vi "Measurement Logic.vi"() -> ()   [LabVIEW 2021, in "Ripple_PMIC.lvlib"]
uses:
  Ripple_PMIC.lvlib
  <vilib>/Plug-In SDKs/Measurements/Measure Call Context/Measure Call Context.lvclass
  Measurement Results.ctl
  Measurement Configuration.ctl
  <instrlib>/niDCPower/nidcpower.llb/niDCPower Output Function.ctl
  <instrlib>/niDCPower/nidcpower.llb/niDCPower Source Mode.ctl
  <instrlib>/niDCPower/nidcpower.llb/niDCPower Wait For Event - Event.ctl
  <instrlib>/niDCPower/nidcpower.llb/niDCPower Measurement Type.ctl
  <instrlib>/niScope/Controls/niScope vertical coupling.ctl
  <instrlib>/niScope/Controls/niScope trigger slope.ctl
  <instrlib>/niScope/Controls/niScope trigger coupling.ctl
  <instrlib>/niScope/Controls/niScope timestamp type.ctl
  <instrlib>/niScope/Configure/Trigger/niScope Configure Trigger Edge.vi
  <instrlib>/niScope/Acquire/Fetch/niScope Fetch WDT.vi
  <vilib>/measure/madcrms.llb/Basic Averaged DC-RMS for 1 Chan.vi
  <vilib>/Plug-In SDKs/Measurements/Measure Call Context/Accessor/Is Canceled.vi
  <instrlib>/niDCPower/nidcpower.llb/niDCPower Get Channel Name From String.vi
  <vilib>/measure/NI_MAPro.lvlib
panel:
  in  "measurement configuration":T1={"Mode of operation"=enum."Perform measurement", "DUT setup time"=0.005, "Aperture time"=0.005, "Source resource name"="", "Source sense"=1009, "Source voltage level"=10.0, "Source current limit"=15.0, "Load resource name"="", "Load sense"=1009, "Load current level"=6.0, "Load voltage limit range"=6.0, "Scope resource name"="", "Scope channel name"="0", "Scope sample rate"=10000.0, "Scope acquisition time"=3.0, "Scope probe attenuation"=1.0} {"Load sense" items=["Local"=1008, "Remote"=1009]; "Source sense" items=["Local"=1008, "Remote"=1009]}
  out "measurement results":T2
  out "measure call context out":refnum<class "Measure Call Context.lvclass">
  in  "measure call context in":refnum<class "Measure Call Context.lvclass">
  out "error out":errorcluster
  in  "error in":errorcluster
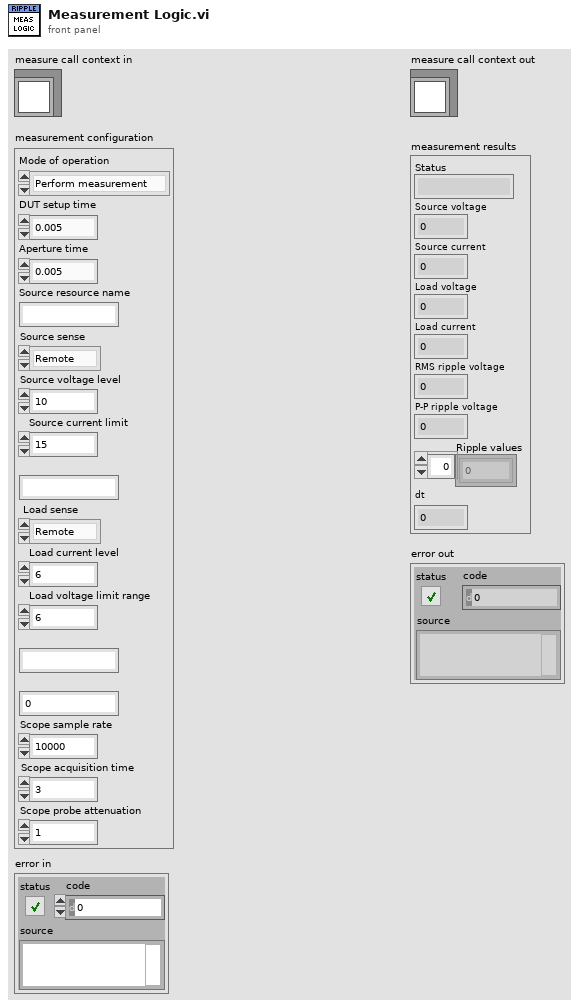
[diagram p1: front panel]
types:
  T1 = typedef "Ripple_PMIC.lvlib/Measurement Configuration.ctl" = cluster{"Mode of operation":enum32{"Power on the DUT", "Perform measurement", "Power off the DUT"}, "DUT setup time":dbl, "Aperture time":dbl, "Source resource name":string, "Source sense":i32, "Source voltage level":dbl, "Source current limit":dbl, "Load resource name":string, "Load sense":i32, "Load current level":dbl, "Load voltage limit range":dbl, "Scope resource name":string, "Scope channel name":string, "Scope sample rate":dbl, "Scope acquisition time":dbl, "Scope probe attenuation":dbl}
  T2 = typedef "Ripple_PMIC.lvlib/Measurement Results.ctl" = cluster{"Status":string, "Source voltage":dbl, "Source current":dbl, "Load voltage":dbl, "Load current":dbl, "RMS ripple voltage":dbl, "P-P ripple voltage":dbl, "Ripple values":dbl[], "dt":dbl}
  T3 = cluster{"Source Session":refnum<k15>, "Load Session":refnum<k15>, "Scope Session":refnum<k15>, "Source channel":string, "Load channel":string}
  T4 = enum32{"Power on the DUT", "Perform measurement", "Power off the DUT"}
  T5 = typedef "niDCPower Wait For Event - Event.ctl" = i32
  T6 = typedef "niDCPower Source Mode.ctl" = i32
  T7 = typedef "niDCPower Output Function.ctl" = i32
  T8 = typedef "niDCPower Measurement Type.ctl" = i32
  T9 = typedef "niScope trigger coupling.ctl" = u16
  T10 = typedef "niScope trigger slope.ctl" = i32
  T11 = typedef "niScope vertical coupling.ctl" = i32
  T12 = typedef "niScope timestamp type.ctl" = i32
  T13 = cluster{"actualSamples":i32, "absoluteInitialX":dbl, "relativeInitialX":dbl, "xIncrement":dbl, "offset":dbl, "gain":dbl, "reserved1":dbl, "reserved2":dbl}
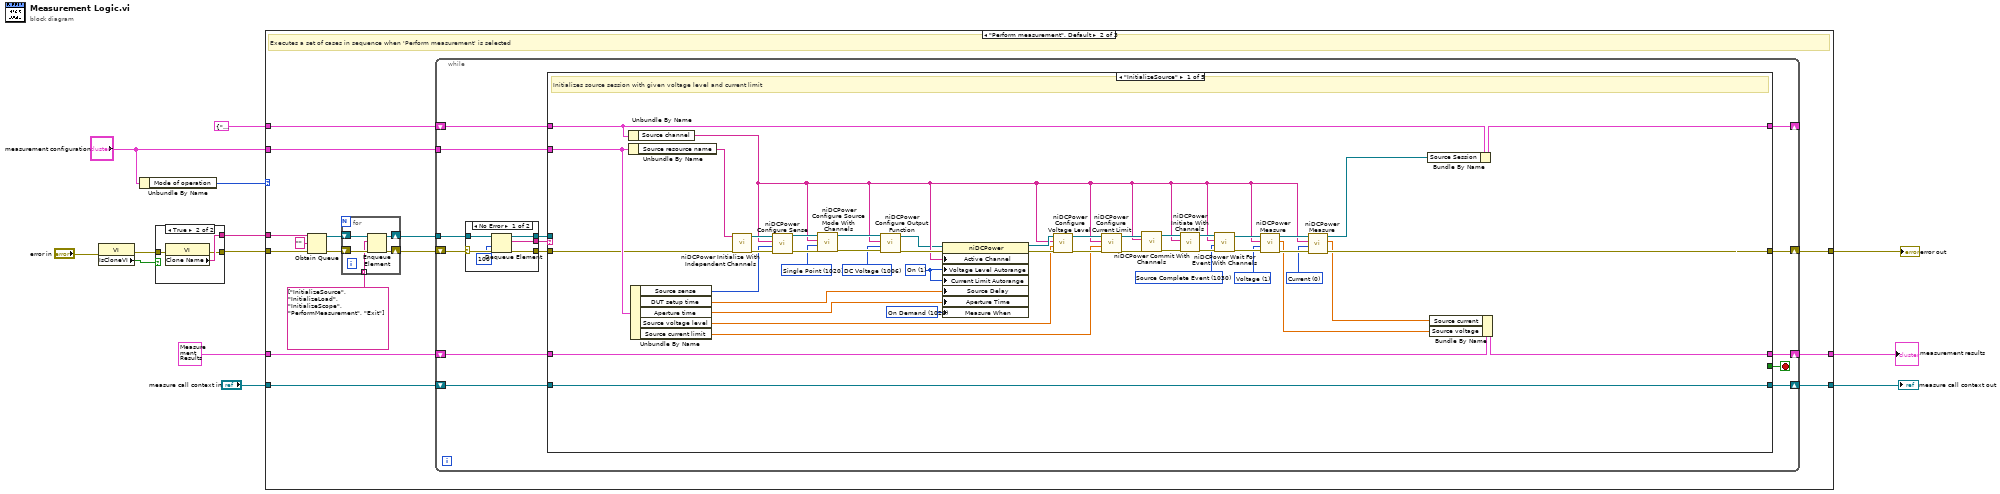
[diagram p0: block diagram]
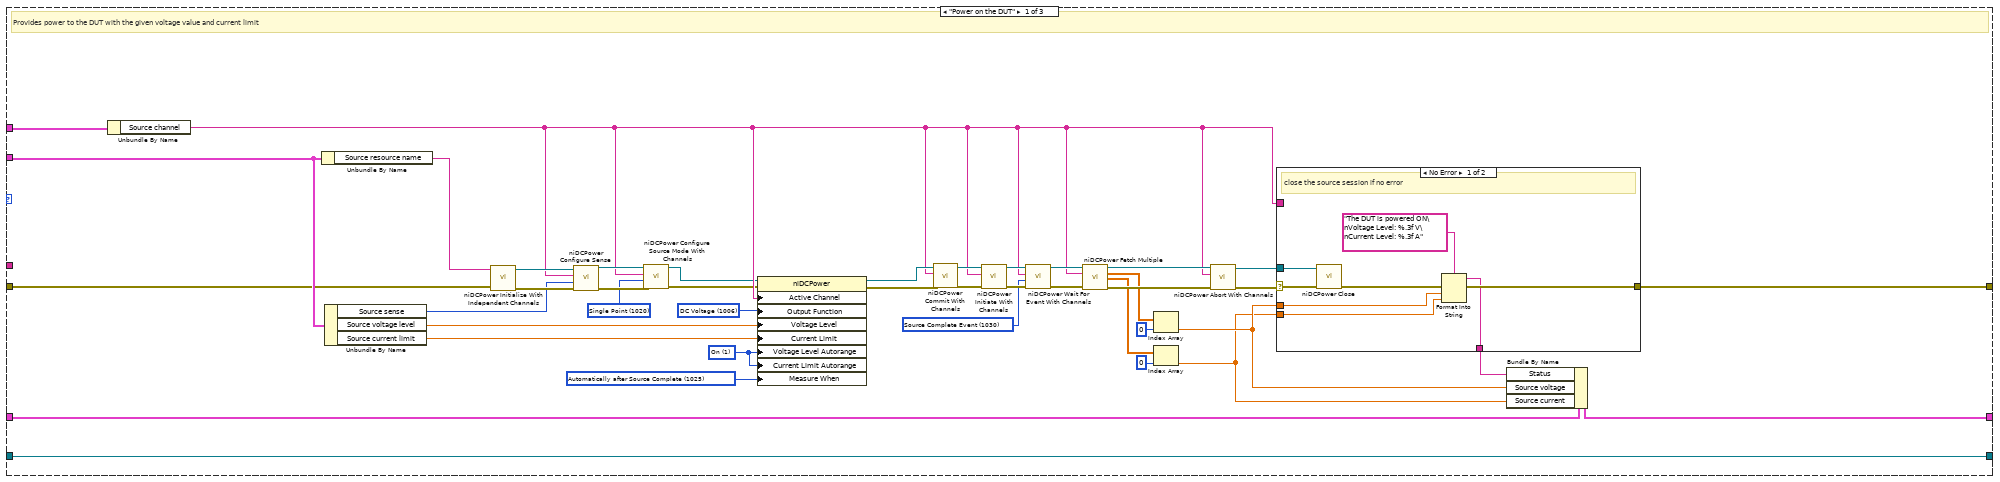
[diagram p2: hidden frame]
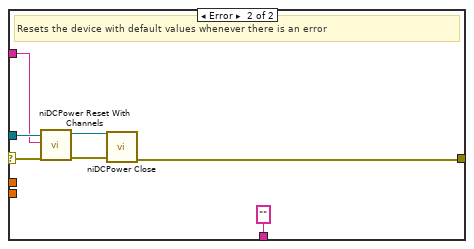
[diagram p3: hidden frame]
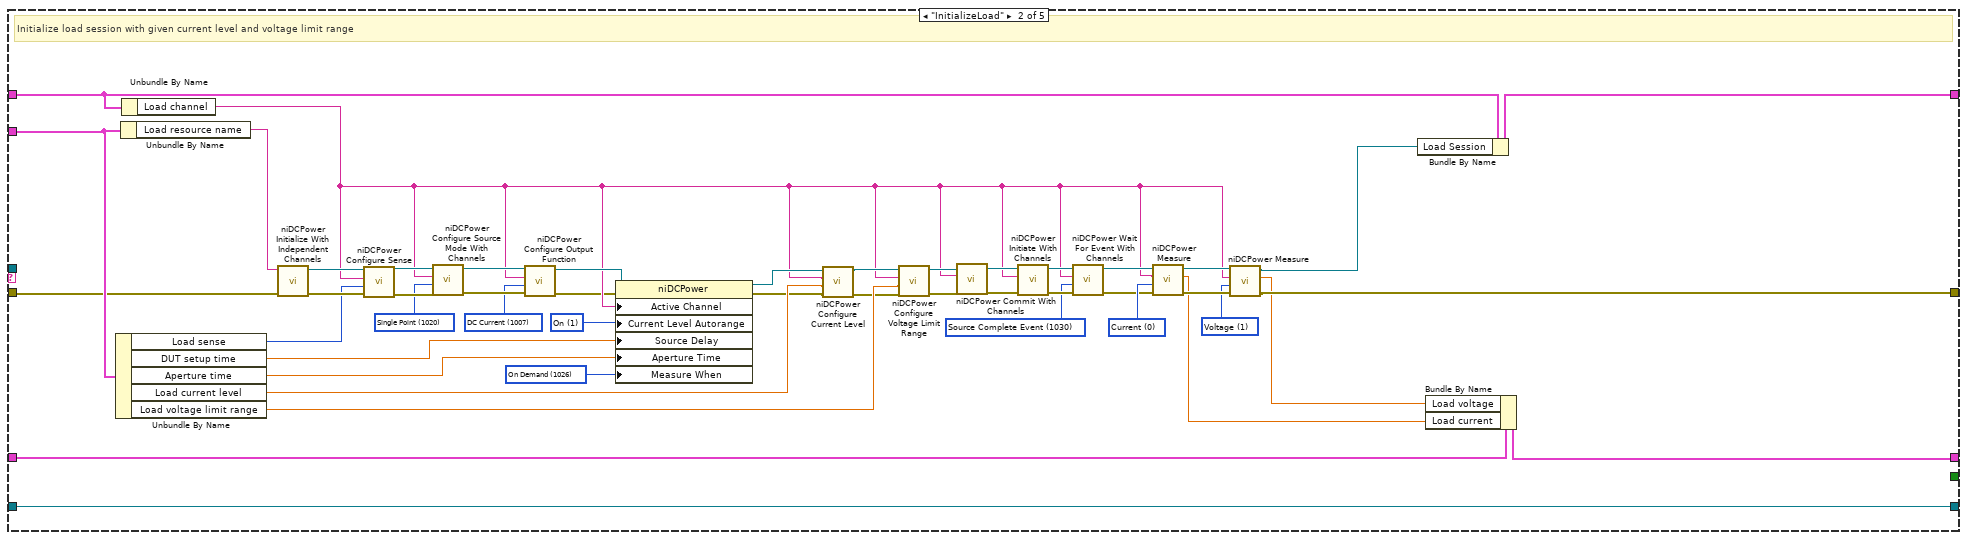
[diagram p4: hidden frame]
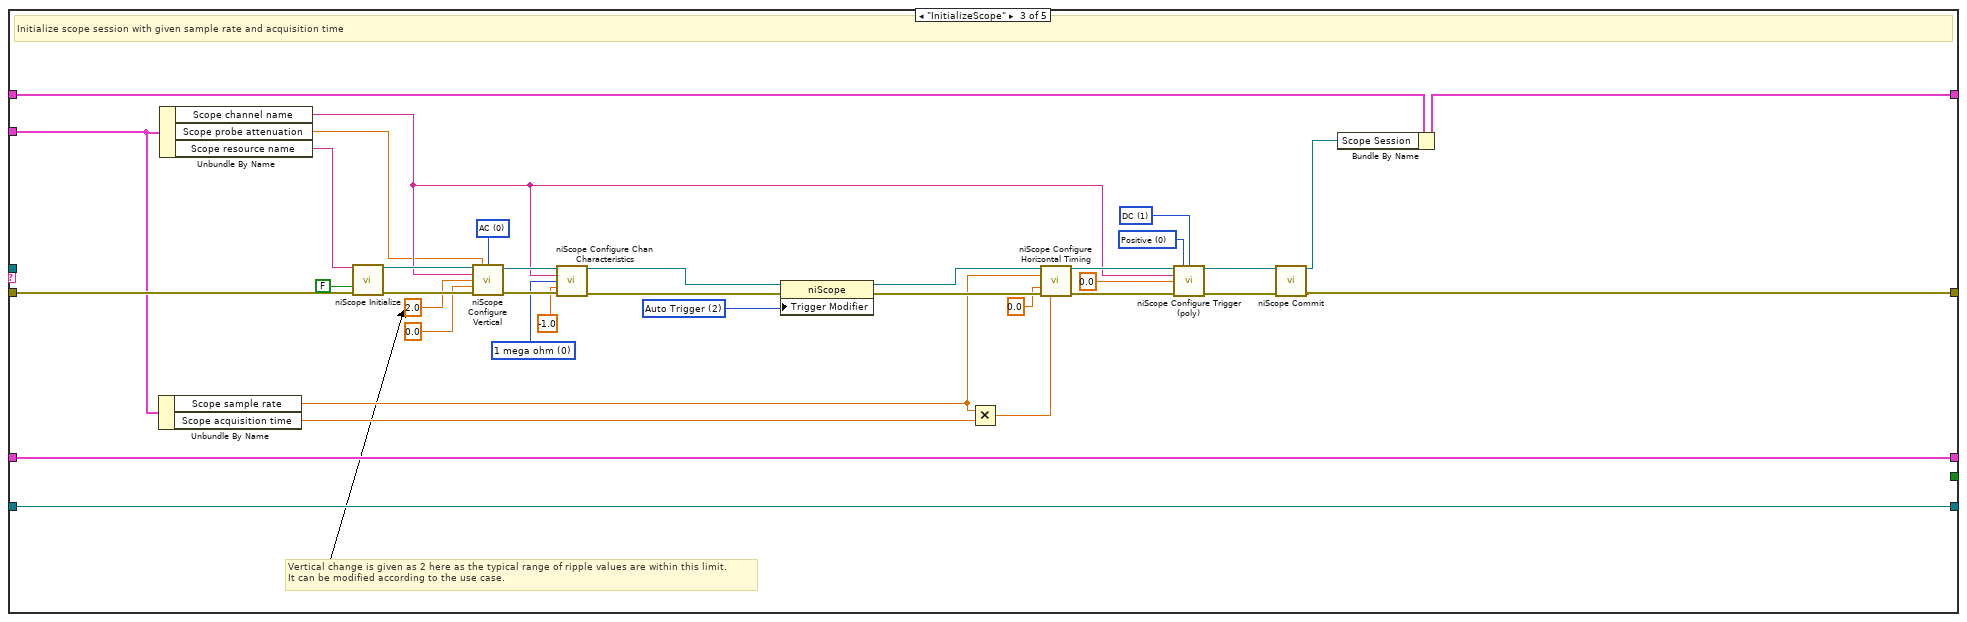
[diagram p5: hidden frame]
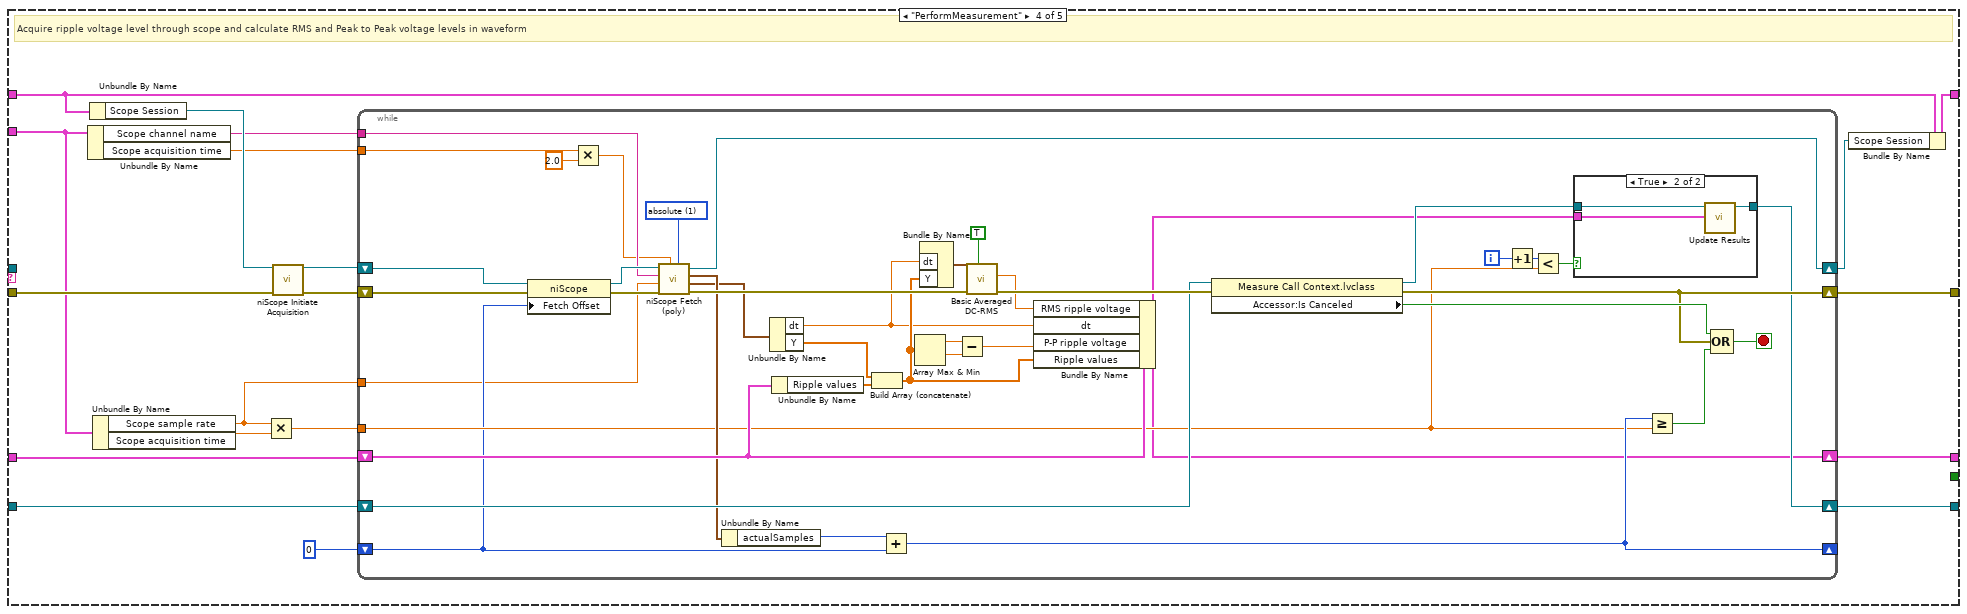
[diagram p6: hidden frame]
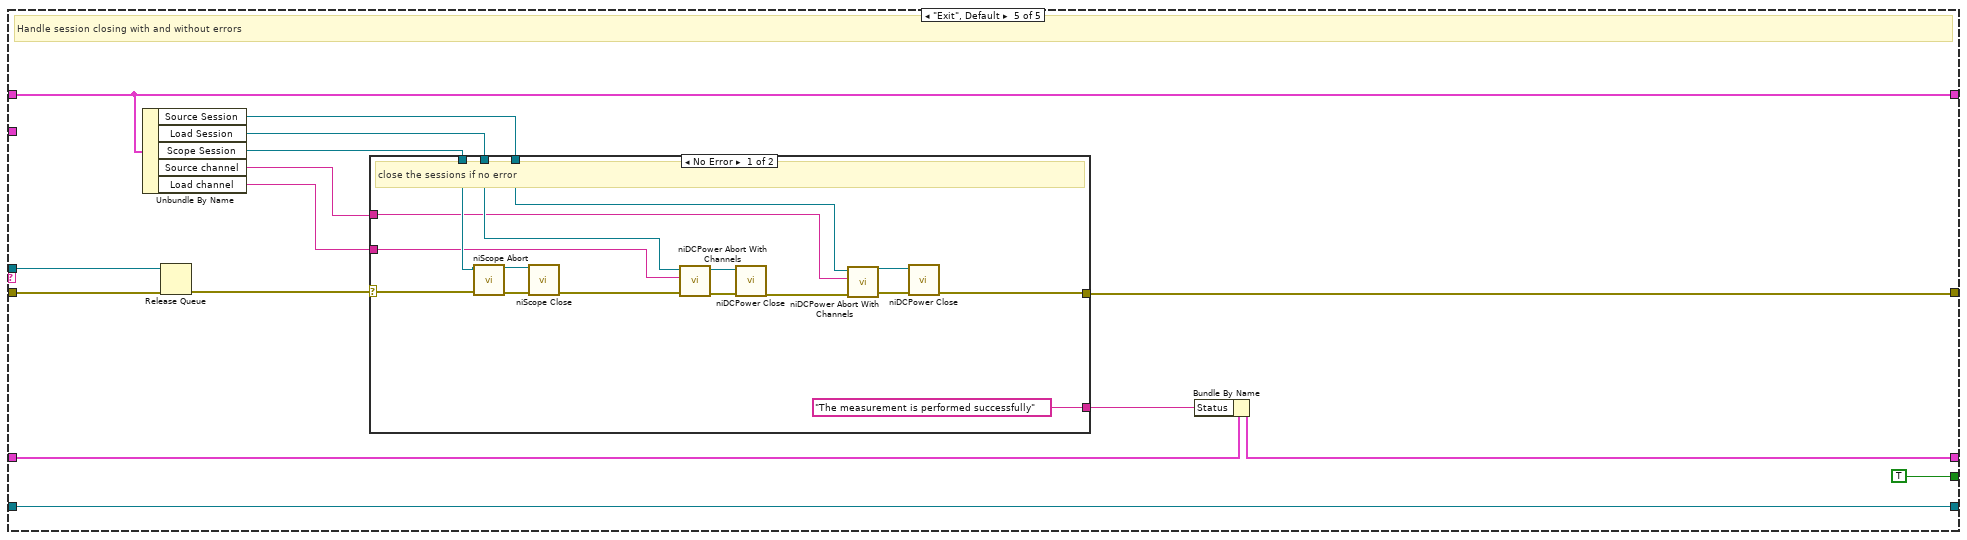
[diagram p8: hidden frame]
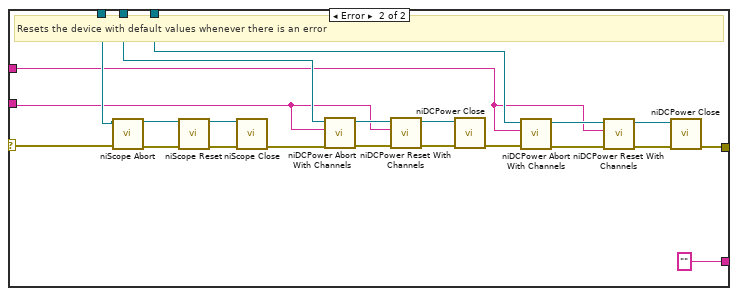
[diagram p9: hidden frame]
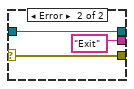
[diagram p10: hidden frame]
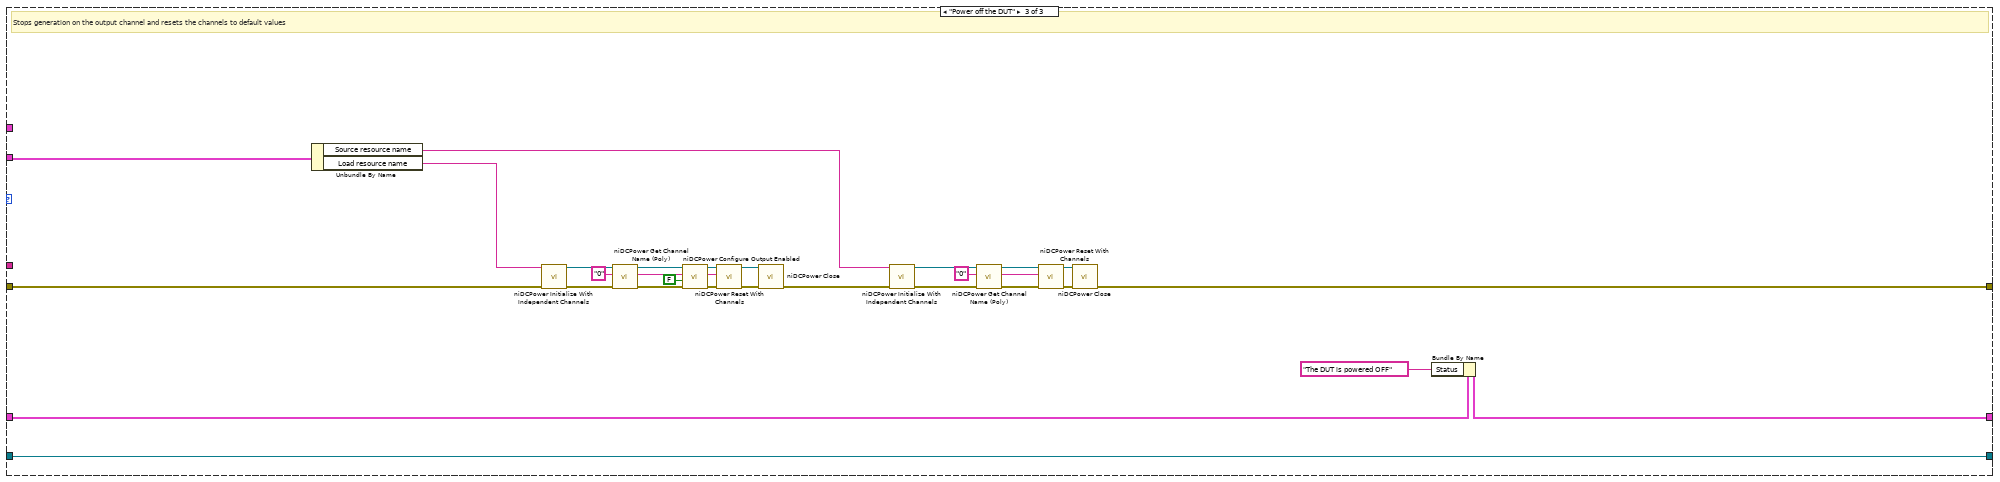
[diagram p11: hidden frame]
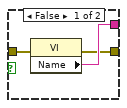
[diagram p12: hidden frame]
diagram:
  n1 = property class="VI"(error in="error in") -> (error out=w12:errorcluster, "IsCloneVI"=w13:bool)  [unwired: 1 in, 1 out]
  n2 = Unbundle By Name("measurement configuration") -> ("Mode of operation"=w6:T4)
  n3 = case shown="True" w13 {
    tunnel: w12 -> [w16 w19]
    tunnel: [w15 w18] -> w4
    tunnel: [w14 w17] -> w5
    frame False {
      n4 = property class="VI"(error in=w16) -> (error out=w14:errorcluster, "Name"=w15:string)  [unwired: 1 in, 1 out]
    }
    frame True {
      n5 = property class="VI"(error in=w19) -> (error out=w17:errorcluster, "Clone Name"=w18:string)  [unwired: 1 in, 1 out]
    }
  }
  n6 = case shown="\"Perform measurement\", Default" w6 {
    tunnel: T3 {"Source Session"="", "Load Session"="", "Scope Session"="", "Source channel"="0", "Load channel"="0"} ("Cluster") -> [w41 w91 _]
    tunnel: T2 {"Status"="", "Source voltage"=0.0, "Source current"=0.0, "Load voltage"=0.0, "Load current"=0.0, "RMS ripple voltage"=0.0, "P-P ripple voltage"=0.0, "Ripple values"=[], "dt"=0.0} ("Measurement Results") -> [w44 w90 w371]
    tunnel: [w39 w89 w375] -> w8
    tunnel: "measurement configuration" -> [w46 w88 w376]
    tunnel: [w45 w87 w370] -> w7
    tunnel: w5 -> [w40 w81 w374]
    tunnel: w4 -> [_ w80 _]
    tunnel: "measure call context in" -> [w22 w78 w368]
    tunnel: [w22 w77 w368] -> w2
    frame "Power on the DUT" {
      w21 = 1025 items=["Automatically after Source Complete"=1025, "On Demand"=1026, "On Measure Trigger"=1027] ("Measurement:Advanced:Measure When")
      w52 = T5 1030 items=["Source Complete Event"=1030, "Measure Complete Event"=1031, "Sequence Iteration Complete Event"=1032, "Sequence Engine Done Event"=1033, "Pulse Complete Event"=1051, "Ready For Pulse Trigger Event"=1052] ("event")
      w26 = 1 items=["Off", "On"] ("Source:DC Voltage:Voltage Level Autorange")
      w59 = T6 1020 items=["Single Point"=1020, "Sequence"=1021] ("source mode")
      w27 = T7 1006 items=["DC Voltage"=1006, "DC Current"=1007, "Pulse Voltage"=1049, "Pulse Current"=1050] ("output function")
      # "Provides power to the DUT with the given voltage value and current limit"
      n7 = Unbundle By Name(w41) -> ("Source channel"=w36:string)
      n8 = Unbundle By Name(w46) -> ("Source resource name"=w51:string)
      n9 = Unbundle By Name(w46) -> ("Source sense"=w20:i32, "Source voltage level"=w24:dbl, "Source current limit"=w25:dbl)
      n10 = call <instrlib>:"niDCPower Initialize With Independent Channels.vi"("error in (no error)"=w40, "resource name"=w51) -> ("error out"=w38:errorcluster, "instrument handle out"=w37:refnum<k15>)  [unwired: 8 in]
      n11 = call <instrlib>:"niDCPower Configure Sense.vi"("error in (no error)"=w38, "sense"=w20, "channel name"=w36, "instrument handle"=w37) -> ("error out"=w60:errorcluster, "instrument handle out"=w61:refnum<k15>)  [unwired: 6 in]
      n12 = call <instrlib>:"niDCPower Configure Source Mode With Channels.vi"("error in (no error)"=w60, "source mode"=w59, "channel name"=w36, "instrument handle"=w61) -> ("error out"=w23:errorcluster, "instrument handle out"=w28:refnum<k15>)  [unwired: 6 in]
      n13 = property class="niDCPower"(reference=w28, error in=w23, "Active Channel"=w36, "Output Function"=w27, "Voltage Level"=w24, "Current Limit"=w25, "Voltage Level Autorange"=w26, "Current Limit Autorange"=w26, "Measure When"=w21) -> (reference out=w58:refnum<k15>, error out=w57:errorcluster)
      n14 = call <instrlib>:"niDCPower Commit With Channels.vi"("error in (no error)"=w57, "channel name"=w36, "instrument handle"=w58) -> ("error out"=w55:errorcluster, "instrument handle out"=w56:refnum<k15>)  [unwired: 7 in]
      n15 = call <instrlib>:"niDCPower Initiate With Channels.vi"("error in (no error)"=w55, "channel name"=w36, "instrument handle"=w56) -> ("error out"=w54:errorcluster, "instrument handle out"=w53:refnum<k15>)  [unwired: 7 in]
      n16 = call <instrlib>:"niDCPower Wait For Event With Channels.vi"("error in (no error)"=w54, "event"=w52, "channel name"=w36, "instrument handle"=w53) -> ("error out"=w49:errorcluster, "instrument handle out"=w50:refnum<k15>)  [unwired: 6 in]
      n17 = call <instrlib>:"niDCPower Fetch Multiple.vi"("instrument handle"=w50, "channel name"=w36, "error in (no error)"=w49) -> ("instrument handle out"=w48:refnum<k15>, "voltage measurements"=w35:dbl[], "current measurements"=w34:dbl[], "error out"=w47:errorcluster)  [unwired: 7 in, 2 out]
      n18 = Index Array(array=w35, index=0) -> (element=w31:dbl)
      n19 = Index Array(array=w34, index=0) -> (element=w30:dbl)
      n20 = call <instrlib>:"niDCPower Abort With Channels.vi"("error in (no error)"=w47, "channel name"=w36, "instrument handle"=w48) -> ("error out"=w43:errorcluster, "instrument handle out"=w42:refnum<k15>)  [unwired: 7 in]
      n21 = case shown="No Error" w43 {
        selector: w43 -> [w68 w75]
        tunnel: w42 -> [w69 w76]
        tunnel: [w66 w72] -> w39
        tunnel: w31 -> [w64 _]
        tunnel: w30 -> [w63 _]
        tunnel: [w62 ""] -> w29
        tunnel: w36 -> [_ w70]
        frame No Error {
          # "close the source session if no error"
          n22 = call <instrlib>:"niDCPower Close.vi"("error in (no error)"=w68, "instrument handle"=w69) -> ("error out"=w65:errorcluster)  [unwired: 9 in]
          n23 = Format Into String(format string="The DUT is powered ON\nVoltage Level: %.3f V\nCurrent Level: %.3f A" ("message"), error in=w65, w64, w63) -> (resulting string=w62:string, error out=w66:errorcluster)  [unwired: 1 in]
        }
        frame Error {
          # "Resets the device with default values whenever there is an error"
          n24 = call <instrlib>:"niDCPower Reset With Channels.vi"("error in (no error)"=w75, "channel name"=w70, "instrument handle"=w76) -> ("error out"=w74:errorcluster, "instrument handle out"=w73:refnum<k15>)  [unwired: 7 in]
          n25 = call <instrlib>:"niDCPower Close.vi"("error in (no error)"=w74, "instrument handle"=w73) -> ("error out"=w72:errorcluster)  [unwired: 9 in]
        }
      }
      n26 = Bundle By Name(cluster=w44, "Status"=w29, "Source voltage"=w31, "Source current"=w30) -> (w45:T2)
    }
    frame "Perform measurement", Default {
      # "Executes a set of cases in sequence when 'Perform measurement' is selected"
      n27 = Obtain Queue(name (unnamed)=w80, element data type="", error in (no error)=w81) -> (queue out=w83:refnum<queue>, error out=w82:errorcluster)  [unwired: 2 in, 1 out]
      n28 = for {
        shift-right: [w94] -> w86
        shift-left: w83 -> [w96]
        shift-right: [w93] -> w85
        shift-left: w82 -> [w95]
        tunnel: string[] ["InitializeSource", "InitializeLoad", "InitializeScope", "PerformMeasurement", "Exit"] ("Step sequence") -> [w92] mode=indexing
        n29 = Enqueue Element(queue=w96, element=w92, error in (no error)=w95) -> (queue out=w94:refnum<queue>, error out=w93:errorcluster)  [unwired: 1 in, 1 out]
      }
      n30 = while {
        tunnel: w88 -> [w107]
        shift-right: [w101] -> _
        shift-left: w91 -> [w102]
        shift-right: [w105] -> w89
        shift-left: w85 -> [w110]
        shift-right: [w103] -> w87
        shift-left: w90 -> [w104]
        tunnel: w86 -> [w109]
        shift-right: [w98] -> w77
        shift-left: w78 -> [w99]
        stop <- w97 stop-if-true
        n31 = case shown="No Error" w110 {
          selector: w110 -> [w362 w366]
          tunnel: w109 -> [w364 w365]
          tunnel: [w363 "Exit" ("t")] -> w108
          tunnel: [w361 w366] -> w106
          tunnel: [w359 w365] -> w100
          frame No Error {
            n32 = Dequeue Element(queue=w364, timeout in ms (-1)=100, error in (no error)=w362) -> (queue out=w359:refnum<queue>, element=w363:string, error out=w361:errorcluster)  [unwired: 1 out]
          }
          frame Error {
          }
        }
        n33 = case shown="\"InitializeSource\"" w108 {
          tunnel: w107 -> [w147 w192 w222 w247 _]
          tunnel: w106 -> [w134 w165 w240 w260 w315]
          tunnel: [w123 w171 w209 w254 w317] -> w105
          tunnel: w102 -> [w120 w168 w219 w244 w312]
          tunnel: [w131 w179 w218 w243 w312] -> w101
          tunnel: w104 -> [w122 w170 w214 w252 w309]
          tunnel: [w121 w169 w214 w253 w308] -> w103
          tunnel: [_ _ _ _ TRUE] -> w97
          tunnel: w100 -> [_ _ _ _ w314]
          tunnel: w99 -> [w118 w164 w207 w251 w306]
          tunnel: [w118 w164 w207 w249 w306] -> w98
          frame "InitializeSource" {
            w112 = 1026 items=["Automatically after Source Complete"=1025, "On Demand"=1026, "On Measure Trigger"=1027] ("Measurement:Advanced:Measure When")
            w125 = T8 0 items=["Current", "Voltage"] ("measurement type")
            w126 = T8 1 items=["Current", "Voltage"] ("measurement type")
            w136 = T5 1030 items=["Source Complete Event"=1030, "Measure Complete Event"=1031, "Sequence Iteration Complete Event"=1032, "Sequence Engine Done Event"=1033, "Pulse Complete Event"=1051, "Ready For Pulse Trigger Event"=1052] ("event")
            w150 = 1 items=["Off", "On"] ("Source:DC Voltage:Voltage Level Autorange")
            w155 = T6 1020 items=["Single Point"=1020, "Sequence"=1021] ("source mode")
            w152 = T7 1006 items=["DC Voltage"=1006, "DC Current"=1007, "Pulse Voltage"=1049, "Pulse Current"=1050] ("output function")
            # "Initializes source session with given voltage level and current limit"
            n34 = Unbundle By Name(w120) -> ("Source channel"=w119:string)
            n35 = Unbundle By Name(w147) -> ("Source resource name"=w135:string)
            n36 = Unbundle By Name(w147) -> ("Source sense"=w111:i32, "DUT setup time"=w114:dbl, "Aperture time"=w113:dbl, "Source voltage level"=w146:dbl, "Source current limit"=w143:dbl)
            n37 = call <instrlib>:"niDCPower Initialize With Independent Channels.vi"("error in (no error)"=w134, "resource name"=w135) -> ("error out"=w132:errorcluster, "instrument handle out"=w133:refnum<k15>)  [unwired: 8 in]
            n38 = call <instrlib>:"niDCPower Configure Sense.vi"("error in (no error)"=w132, "sense"=w111, "channel name"=w119, "instrument handle"=w133) -> ("error out"=w156:errorcluster, "instrument handle out"=w157:refnum<k15>)  [unwired: 6 in]
            n39 = call <instrlib>:"niDCPower Configure Source Mode With Channels.vi"("error in (no error)"=w156, "source mode"=w155, "channel name"=w119, "instrument handle"=w157) -> ("error out"=w153:errorcluster, "instrument handle out"=w154:refnum<k15>)  [unwired: 6 in]
            n40 = call <instrlib>:"niDCPower Configure Output Function.vi"("error in (no error)"=w153, "output function"=w152, "channel name"=w119, "instrument handle"=w154) -> ("error out"=w151:errorcluster, "instrument handle out"=w115:refnum<k15>)  [unwired: 6 in]
            n41 = property class="niDCPower"(reference=w115, error in=w151, "Active Channel"=w119, "Voltage Level Autorange"=w150, "Current Limit Autorange"=w150, "Source Delay"=w114, "Aperture Time"=w113, "Measure When"=w112) -> (reference out=w149:refnum<k15>, error out=w148:errorcluster)
            n42 = call <instrlib>:"niDCPower Configure Voltage Level.vi"("error in (no error)"=w148, "voltage level"=w146, "channel name"=w119, "instrument handle"=w149) -> ("error out"=w144:errorcluster, "instrument handle out"=w145:refnum<k15>)  [unwired: 6 in]
            n43 = call <instrlib>:"niDCPower Configure Current Limit.vi"("error in (no error)"=w144, "current limit"=w143, "channel name"=w119, "instrument handle"=w145) -> ("error out"=w142:errorcluster, "instrument handle out"=w141:refnum<k15>)  [unwired: 6 in]
            n44 = call <instrlib>:"niDCPower Commit With Channels.vi"("error in (no error)"=w142, "channel name"=w119, "instrument handle"=w141) -> ("error out"=w139:errorcluster, "instrument handle out"=w140:refnum<k15>)  [unwired: 7 in]
            n45 = call <instrlib>:"niDCPower Initiate With Channels.vi"("error in (no error)"=w139, "channel name"=w119, "instrument handle"=w140) -> ("error out"=w138:errorcluster, "instrument handle out"=w137:refnum<k15>)  [unwired: 7 in]
            n46 = call <instrlib>:"niDCPower Wait For Event With Channels.vi"("error in (no error)"=w138, "event"=w136, "channel name"=w119, "instrument handle"=w137) -> ("error out"=w129:errorcluster, "instrument handle out"=w130:refnum<k15>)  [unwired: 6 in]
            n47 = call <instrlib>:"niDCPower Measure.vi"("error in (no error)"=w129, "measurement type"=w126, "channel name"=w119, "instrument handle"=w130) -> ("error out"=w127:errorcluster, "measurement"=w116:dbl, "instrument handle out"=w128:refnum<k15>)  [unwired: 5 in]
            n48 = call <instrlib>:"niDCPower Measure.vi"("error in (no error)"=w127, "measurement type"=w125, "channel name"=w119, "instrument handle"=w128) -> ("error out"=w123:errorcluster, "measurement"=w117:dbl, "instrument handle out"=w124:refnum<k15>)  [unwired: 5 in]
            n49 = Bundle By Name(cluster=w120, "Source Session"=w124) -> (w131:T3)
            n50 = Bundle By Name(cluster=w122, "Source current"=w117, "Source voltage"=w116) -> (w121:T2)
          }
          frame "InitializeLoad" {
            w159 = 1026 items=["Automatically after Source Complete"=1025, "On Demand"=1026, "On Measure Trigger"=1027] ("Measurement:Advanced:Measure When")
            w175 = T8 1 items=["Current", "Voltage"] ("measurement type")
            w176 = T8 0 items=["Current", "Voltage"] ("measurement type")
            w193 = T5 1030 items=["Source Complete Event"=1030, "Measure Complete Event"=1031, "Sequence Iteration Complete Event"=1032, "Sequence Engine Done Event"=1033, "Pulse Complete Event"=1051, "Ready For Pulse Trigger Event"=1052] ("event")
            w198 = 1 items=["Off", "On"] ("Source:DC Voltage:Voltage Level Autorange")
            w202 = T6 1020 items=["Single Point"=1020, "Sequence"=1021] ("source mode")
            w199 = T7 1007 items=["DC Voltage"=1006, "DC Current"=1007, "Pulse Voltage"=1049, "Pulse Current"=1050] ("output function")
            # "Initialize load session with given current level and voltage limit range"
            n51 = Unbundle By Name(w192) -> ("Load sense"=w158:i32, "DUT setup time"=w161:dbl, "Aperture time"=w160:dbl, "Load current level"=w189:dbl, "Load voltage limit range"=w184:dbl)
            n52 = Unbundle By Name(w192) -> ("Load resource name"=w182:string)
            n53 = Unbundle By Name(w168) -> ("Load channel"=w167:string)
            n54 = call <instrlib>:"niDCPower Initialize With Independent Channels.vi"("error in (no error)"=w165, "resource name"=w182) -> ("error out"=w180:errorcluster, "instrument handle out"=w181:refnum<k15>)  [unwired: 8 in]
            n55 = call <instrlib>:"niDCPower Configure Sense.vi"("error in (no error)"=w180, "sense"=w158, "channel name"=w167, "instrument handle"=w181) -> ("error out"=w203:errorcluster, "instrument handle out"=w204:refnum<k15>)  [unwired: 6 in]
            n56 = call <instrlib>:"niDCPower Configure Source Mode With Channels.vi"("error in (no error)"=w203, "source mode"=w202, "channel name"=w167, "instrument handle"=w204) -> ("error out"=w200:errorcluster, "instrument handle out"=w201:refnum<k15>)  [unwired: 6 in]
            n57 = call <instrlib>:"niDCPower Configure Output Function.vi"("error in (no error)"=w200, "output function"=w199, "channel name"=w167, "instrument handle"=w201) -> ("error out"=w166:errorcluster, "instrument handle out"=w191:refnum<k15>)  [unwired: 6 in]
            n58 = property class="niDCPower"(reference=w191, error in=w166, "Active Channel"=w167, "Current Level Autorange"=w198, "Source Delay"=w161, "Aperture Time"=w160, "Measure When"=w159) -> (reference out=w190:refnum<k15>, error out=w188:errorcluster)
            n59 = call <instrlib>:"niDCPower Configure Current Level.vi"("error in (no error)"=w188, "current level"=w189, "channel name"=w167, "instrument handle"=w190) -> ("error out"=w183:errorcluster, "instrument handle out"=w185:refnum<k15>)  [unwired: 6 in]
            n60 = call <instrlib>:"niDCPower Configure Voltage Limit Range.vi"("error in (no error)"=w183, "voltage limit range"=w184, "channel name"=w167, "instrument handle"=w185) -> ("error out"=w187:errorcluster, "instrument handle out"=w186:refnum<k15>)  [unwired: 6 in]
            n61 = call <instrlib>:"niDCPower Commit With Channels.vi"("error in (no error)"=w187, "channel name"=w167, "instrument handle"=w186) -> ("error out"=w196:errorcluster, "instrument handle out"=w197:refnum<k15>)  [unwired: 7 in]
            n62 = call <instrlib>:"niDCPower Initiate With Channels.vi"("error in (no error)"=w196, "channel name"=w167, "instrument handle"=w197) -> ("error out"=w195:errorcluster, "instrument handle out"=w194:refnum<k15>)  [unwired: 7 in]
            n63 = call <instrlib>:"niDCPower Wait For Event With Channels.vi"("error in (no error)"=w195, "event"=w193, "channel name"=w167, "instrument handle"=w194) -> ("error out"=w173:errorcluster, "instrument handle out"=w174:refnum<k15>)  [unwired: 6 in]
            n64 = call <instrlib>:"niDCPower Measure.vi"("error in (no error)"=w173, "measurement type"=w176, "channel name"=w167, "instrument handle"=w174) -> ("error out"=w177:errorcluster, "measurement"=w163:dbl, "instrument handle out"=w178:refnum<k15>)  [unwired: 5 in]
            n65 = call <instrlib>:"niDCPower Measure.vi"("error in (no error)"=w177, "measurement type"=w175, "channel name"=w167, "instrument handle"=w178) -> ("error out"=w171:errorcluster, "measurement"=w162:dbl, "instrument handle out"=w172:refnum<k15>)  [unwired: 5 in]
            n66 = Bundle By Name(cluster=w168, "Load Session"=w172) -> (w179:T3)
            n67 = Bundle By Name(cluster=w170, "Load voltage"=w162, "Load current"=w163) -> (w169:T2)
          }
          frame "InitializeScope" {
            w227 = T9 1 items=["AC"=0, "DC"=1, "HF Reject"=3, "LF Reject"=4, "AC Plus HF Reject"=1001] ("trigger coupling")
            w208 = T10 0 items=["Positive", "Negative"] ("trigger slope")
            w228 = 2 items=["None"=1, "Auto Trigger"=2] ("Triggering:Trigger Modifier")
            w232 = u32 0 items=["1 mega ohm"=0, "50 ohms"=2] ("input impedance")
            w235 = T11 0 items=["AC", "DC", "Ground"] ("vertical coupling")
            # "Vertical change is given as 2 here as the typical range of ripple values are within this limit.\nIt can be modified according to the use case."
            # "Initialize scope session with given sample rate and acquisition time"
            n68 = Unbundle By Name(w222) -> ("Scope sample rate"=w212:dbl, "Scope acquisition time"=w211:dbl)
            n69 = Unbundle By Name(w222) -> ("Scope channel name"=w213:string, "Scope probe attenuation"=w206:dbl, "Scope resource name"=w205:string)
            n70 = call <instrlib>:"niScope Initialize.vi"("resource name"=w205, "reset device"=FALSE, "error in"=w240) -> ("instrument handle"=w239:refnum<k15>, "error out"=w238:errorcluster)  [unwired: 11 in]
            n71 = call <instrlib>:"niScope Configure Vertical.vi"("instrument handle"=w239, "probe attenuation"=w206, "vertical coupling"=w235, "channels"=w213, "vertical range"=2.0, "vertical offset"=0.0, "error in"=w238) -> ("instrument handle out"=w234:refnum<k15>, "error out"=w233:errorcluster)  [unwired: 7 in]
            n72 = call <instrlib>:"niScope Configure Chan Characteristics.vi"("instrument handle"=w234, "channels"=w213, "input impedance"=w232, "maximum input frequency"=-1.0, "error in"=w233) -> ("instrument handle out"=w230:refnum<k15>, "error out"=w229:errorcluster)  [unwired: 9 in]
            n73 = property class="niScope"(reference=w230, error in=w229, "Trigger Modifier"=w228) -> (reference out=w226:refnum<k15>, error out=w225:errorcluster)
            n74 = Multiply(x=w212, y=w211) -> (x*y=w210:dbl)
            n75 = call <instrlib>:"niScope Configure Horizontal Timing.vi"("instrument handle"=w226, "min sample rate"=w212, "reference position"=0.0, "error in"=w225, "min record length"=w210) -> ("instrument handle out"=w224:refnum<k15>, "error out"=w223:errorcluster)  [unwired: 9 in]
            n76 = call-poly <instrlib>:"niScope Configure Trigger (poly).vi"("instrument handle"=w224, "trigger slope"=w208, "trigger coupling"=w227, "trigger source"=w213, "trigger level"=0.0, "error in"=w223) -> ("instrument handle out"=w217:refnum<k15>, "error out"=w216:errorcluster)  [unwired: 8 in]
            n77 = call <instrlib>:"niScope Commit.vi"("instrument handle"=w217, "error in"=w216) -> ("instrument handle out"=w215:refnum<k15>, "error out"=w209:errorcluster)  [unwired: 12 in]
            n78 = Bundle By Name(cluster=w219, "Scope Session"=w215) -> (w218:T3)
          }
          frame "PerformMeasurement" {
            # "Acquire ripple voltage level through scope and calculate RMS and Peak to Peak voltage levels in waveform"
            n79 = Unbundle By Name(w247) -> ("Scope channel name"=w246:string, "Scope acquisition time"=w242:dbl)
            n80 = Unbundle By Name(w244) -> ("Scope Session"=w259:refnum<k15>)
            n81 = Unbundle By Name(w247) -> ("Scope sample rate"=w248:dbl, "Scope acquisition time"=w256:dbl)
            n82 = Multiply(x=w248, y=w256) -> (x*y=w255:dbl)
            n83 = call <instrlib>:"niScope Initiate Acquisition.vi"("instrument handle"=w259, "error in"=w260) -> ("instrument handle out"=w257:refnum<k15>, "error out"=w258:errorcluster)  [unwired: 12 in]
            n84 = while {
              shift-right: [w297] -> w254
              shift-left: w258 -> [w281]
              shift-right: [w270] -> w253
              shift-left: w252 -> [w289]
              shift-right: [w293] -> w249
              shift-left: w251 -> [w295]
              tunnel: w255 -> [w284]
              shift-right: [w268] -> w245
              shift-left: w257 -> [w282]
              shift-right: [w285] -> _
              shift-left: 0 -> [w283]
              tunnel: w248 -> [w277]
              tunnel: w246 -> [w269]
              tunnel: w242 -> [w263]
              i -> [w291]
              stop <- w275 stop-if-true
              w301 = T12 1 items=["relative", "absolute"] ("timestamp Type")
              n85 = property class="niScope"(reference=w282, error in=w281, "Fetch Offset"=w283) -> (reference out=w279:refnum<k15>, error out=w280:errorcluster)
              n86 = Multiply(x=w263, y=2.0) -> (x*y=w262:dbl)
              n87 = call-poly <instrlib>:"niScope Fetch (poly).vi"("timestamp Type"=w301, "timeout"=w262, "error in"=w280, "numSamples"=w277, "channels"=w269, "instrument handle"=w279) -> ("error out"=w300:errorcluster, "wfm"=w278:waveform(dbl), "wfm info"=w288:T13, "instrument handle out"=w268:refnum<k15>)  [unwired: 2 in]
              n88 = Unbundle By Name(w288) -> ("actualSamples"=w287:i32)
              n89 = Unbundle By Name(w278) -> ("dt"=w266:dbl, "Y"=w272:dbl[])
              n90 = Unbundle By Name(w289) -> ("Ripple values"=w276:dbl[])
              n91 = Build Array (concatenate)(w272, w276) -> (w267:dbl[])
              n92 = Add(x=w287, y=w283) -> (x+y=w285:i32)
              n93 = Array Max & Min(array=w267) -> (max value=w274:dbl, min value=w273:dbl)  [unwired: 2 out]
              n94 = Bundle By Name("dt"=w266, "Y"=w267) -> (w265:waveform(dbl))  [unwired: 1 in]
              n95 = Subtract(x=w274, y=w273) -> (x-y=w299:dbl)
              n96 = call-poly <vilib>:"Basic Averaged DC-RMS.vi"("reset"=TRUE, "error in (no error)"=w300, "signal in"=w265) -> ("error out"=w296:errorcluster, "RMS value"=w271:dbl)  [unwired: 5 in, 2 out]
              n97 = Bundle By Name(cluster=w289, "RMS ripple voltage"=w271, "dt"=w266, "P-P ripple voltage"=w299, "Ripple values"=w267) -> (w270:T2)
              n98 = property class="Measure Call Context.lvclass"(reference=w295, error in=w296) -> (reference out=w294:refnum<class "Measure Call Context.lvclass">, error out=w297:errorcluster, "Accessor:Is Canceled"=w298:bool)
              n99 = Increment(x=w291) -> (x+1=w292:i32)
              n100 = Less?(x=w292, y=w284) -> (x < y?=w290:bool)
              n101 = case shown="True" w290 {
                tunnel: [w302 w305] -> w293
                tunnel: w294 -> [w302 w304]
                tunnel: w270 -> [_ w303]
                frame False {
                }
                frame True {
                  n102 = call <vilib>:"Update Results.vi"("measurement results"=w303, "measure call context in"=w304) -> ("measure call context out"=w305:refnum<class "Measure Call Context.lvclass">)  [unwired: 8 in, 1 out]
                }
              }
              n103 = Greater Or Equal?(x=w285, y=w284) -> (x >= y?=w286:bool)
              n104 = Compound Arithmetic op=OR(w298, w297, w286) -> (w275:bool)
            }
            n105 = Bundle By Name(cluster=w244, "Scope Session"=w245) -> (w243:T3)
          }
          frame "Exit", Default {
            # "Handle session closing with and without errors"
            n106 = Unbundle By Name(w312) -> ("Source Session"=w320:refnum<k15>, "Load Session"=w319:refnum<k15>, "Scope Session"=w318:refnum<k15>, "Source channel"=w311:string, "Load channel"=w310:string)
            n107 = Release Queue(queue=w314, error in (no error)=w315) -> (error out=w313:errorcluster)  [unwired: 1 in, 2 out]
            n108 = case shown="No Error" w313 {
              selector: w313 -> [w329 w357]
              tunnel: w320 -> [w321 w339]
              tunnel: w319 -> [w325 w340]
              tunnel: w318 -> [w336 w358]
              tunnel: [w324 w342] -> w317
              tunnel: w311 -> [w322 w337]
              tunnel: w310 -> [w328 w338]
              tunnel: ["The measurement is performed successfully" ("Status") "" ("Status")] -> w307
              frame No Error {
                # "close the sessions if no error"
                n109 = call <instrlib>:"niScope Abort.vi"("instrument handle"=w336, "error in"=w329) -> ("instrument handle out"=w333:refnum<k15>, "error out"=w332:errorcluster)  [unwired: 12 in]
                n110 = call <instrlib>:"niScope Close.vi"("instrument handle"=w333, "error in"=w332) -> ("error out"=w326:errorcluster)  [unwired: 13 in]
                n111 = call <instrlib>:"niDCPower Abort With Channels.vi"("error in (no error)"=w326, "channel name"=w328, "instrument handle"=w325) -> ("error out"=w330:errorcluster, "instrument handle out"=w331:refnum<k15>)  [unwired: 7 in]
                n112 = call <instrlib>:"niDCPower Close.vi"("error in (no error)"=w330, "instrument handle"=w331) -> ("error out"=w323:errorcluster)  [unwired: 9 in]
                n113 = call <instrlib>:"niDCPower Abort With Channels.vi"("error in (no error)"=w323, "channel name"=w322, "instrument handle"=w321) -> ("error out"=w334:errorcluster, "instrument handle out"=w335:refnum<k15>)  [unwired: 7 in]
                n114 = call <instrlib>:"niDCPower Close.vi"("error in (no error)"=w334, "instrument handle"=w335) -> ("error out"=w324:errorcluster)  [unwired: 9 in]
              }
              frame Error {
                # "Resets the device with default values whenever there is an error"
                n115 = call <instrlib>:"niScope Abort.vi"("instrument handle"=w358, "error in"=w357) -> ("instrument handle out"=w348:refnum<k15>, "error out"=w347:errorcluster)  [unwired: 12 in]
                n116 = call <instrlib>:"niScope Reset.vi"("instrument handle"=w348, "error in"=w347) -> ("instrument handle out"=w346:refnum<k15>, "error out"=w345:errorcluster)  [unwired: 12 in]
                n117 = call <instrlib>:"niScope Close.vi"("instrument handle"=w346, "error in"=w345) -> ("error out"=w343:errorcluster)  [unwired: 13 in]
                n118 = call <instrlib>:"niDCPower Abort With Channels.vi"("error in (no error)"=w343, "channel name"=w338, "instrument handle"=w340) -> ("error out"=w351:errorcluster, "instrument handle out"=w352:refnum<k15>)  [unwired: 7 in]
                n119 = call <instrlib>:"niDCPower Reset With Channels.vi"("error in (no error)"=w351, "channel name"=w338, "instrument handle"=w352) -> ("error out"=w350:errorcluster, "instrument handle out"=w349:refnum<k15>)  [unwired: 7 in]
                n120 = call <instrlib>:"niDCPower Close.vi"("error in (no error)"=w350, "instrument handle"=w349) -> ("error out"=w341:errorcluster)  [unwired: 9 in]
                n121 = call <instrlib>:"niDCPower Abort With Channels.vi"("error in (no error)"=w341, "channel name"=w337, "instrument handle"=w339) -> ("error out"=w354:errorcluster, "instrument handle out"=w356:refnum<k15>)  [unwired: 7 in]
                n122 = call <instrlib>:"niDCPower Reset With Channels.vi"("error in (no error)"=w354, "channel name"=w337, "instrument handle"=w356) -> ("error out"=w353:errorcluster, "instrument handle out"=w355:refnum<k15>)  [unwired: 7 in]
                n123 = call <instrlib>:"niDCPower Close.vi"("error in (no error)"=w353, "instrument handle"=w355) -> ("error out"=w342:errorcluster)  [unwired: 9 in]
              }
            }
            n124 = Bundle By Name(cluster=w309, "Status"=w307) -> (w308:T2)
          }
        }
      }
    }
    frame "Power off the DUT" {
      # "Stops generation on the output channel and resets the channels to default values"
      n125 = Unbundle By Name(w376) -> ("Source resource name"=w378:string, "Load resource name"=w381:string)
      n126 = call <instrlib>:"niDCPower Initialize With Independent Channels.vi"("error in (no error)"=w374, "resource name"=w381) -> ("error out"=w382:errorcluster, "instrument handle out"=w380:refnum<k15>)  [unwired: 8 in]
      n127 = call-poly <instrlib>:"niDCPower Get Channel Name (Poly).vi"("error in (no error)"=w382, "index"="0", "instrument handle"=w380) -> ("error out"=w389:errorcluster, "name"=w387:string, "instrument handle out"=w388:refnum<k15>)  [unwired: 6 in]
      n128 = call <instrlib>:"niDCPower Configure Output Enabled.vi"("error in (no error)"=w389, "output enabled"=FALSE, "channel name"=w387, "instrument handle"=w388) -> ("error out"=w396:errorcluster, "instrument handle out"=w395:refnum<k15>)  [unwired: 6 in]
      n129 = call <instrlib>:"niDCPower Reset With Channels.vi"("error in (no error)"=w396, "channel name"=w387, "instrument handle"=w395) -> ("error out"=w390:errorcluster, "instrument handle out"=w391:refnum<k15>)  [unwired: 7 in]
      n130 = call <instrlib>:"niDCPower Close.vi"("error in (no error)"=w390, "instrument handle"=w391) -> ("error out"=w385:errorcluster)  [unwired: 9 out]
      n131 = call <instrlib>:"niDCPower Initialize With Independent Channels.vi"("error in (no error)"=w385, "resource name"=w378) -> ("error out"=w379:errorcluster, "instrument handle out"=w377:refnum<k15>)  [unwired: 8 in]
      n132 = call-poly <instrlib>:"niDCPower Get Channel Name (Poly).vi"("error in (no error)"=w379, "index"="0", "instrument handle"=w377) -> ("error out"=w384:errorcluster, "name"=w383:string, "instrument handle out"=w386:refnum<k15>)  [unwired: 6 in]
      n133 = call <instrlib>:"niDCPower Reset With Channels.vi"("error in (no error)"=w384, "channel name"=w383, "instrument handle"=w386) -> ("error out"=w393:errorcluster, "instrument handle out"=w392:refnum<k15>)  [unwired: 7 in]
      n134 = call <instrlib>:"niDCPower Close.vi"("error in (no error)"=w393, "instrument handle"=w392) -> ("error out"=w375:errorcluster)  [unwired: 9 out]
      n135 = Bundle By Name(cluster=w371, "Status"="The DUT is powered OFF") -> (w370:T2)
    }
  }
  "error out" <- w8
  "measure call context out" <- w2
  "measurement results" <- w7
